vi "2636 EPSC Custom Pulse Sweep.vi"() -> ()   [LabVIEW 2023]
uses:
  <instrlib>/Keithley 2600 Series/Public/Channel.ctl
  <instrlib>/Keithley 2600 Series/Keithley 2600 Series.lvlib
  <userlib>/_OpenG.lib/time/time.llb/openg_time.lvlib
panel:
  out "Pulse Level Size":i32
  in  "Pulse Levels (V)":dbl[](array[numeric])=[1.0, 2.0, 4.0]
  in  "error in (no error)":errorcluster
  in  "Log Time After Pulses (s)":dbl=0.5 format="%#_13g"
  in  "Log Time Before Pulses (s)":dbl=0.5 format="%#_13g"
  in  "Auto Enable Output":bool=TRUE
  in  "Reset":bool=TRUE
  in  "Error Query":bool
  out "Pulsed IV Filename Out":path caption="Filename Out"
  in  "Pulsed IV Filename":path=path "C:/Data/pulse_I_V.lvm" caption="Filename"
  out "Pulse IV":cluster{"X":dbl[], "Y":dbl[]}[](graph)
  out "I_ds Log Filename Out":path caption="Filename Out"
  in  "I_ds Log Filename":path=path "C:/Data/I_ds_vs_time.lvm" caption="Filename"
  out "Data":dbl[](array[numeric])
  out "Result Chart":dynamicdata(graph)
  out "error out":errorcluster
  out "Complete?":bool
  out "Overflow?":bool
  in  "Stop":bool
  in  "Pulse Duration (s)":dbl=0.01
  in  "Post-Pulse Duration (s)":dbl=0.05
  in  "Pre-Pulse Duration (s)":dbl=0.05
  in  "Buffer size":u32=1024
  in  "Drain Source Channel":T1=enum."Channel B"
  in  "V_ds(V)":dbl=0.01
  in  "I_ds NPLC":dbl=0.1
  in  "I_ds Range (A)":dbl=1e-06
  in  "I pulse Range (A)":dbl=1e-06
  in  "I pulse NPLC":dbl=0.1
  in  "Pulse Channel":T1
  in  "2636 Address":refnum<visa-resource-name>="GPIB0::26::INSTR"
  # "Synaptic EPSC Custom Pulse Sweep (Three-terminal Devices)"
  # "by JHC (20250322)"
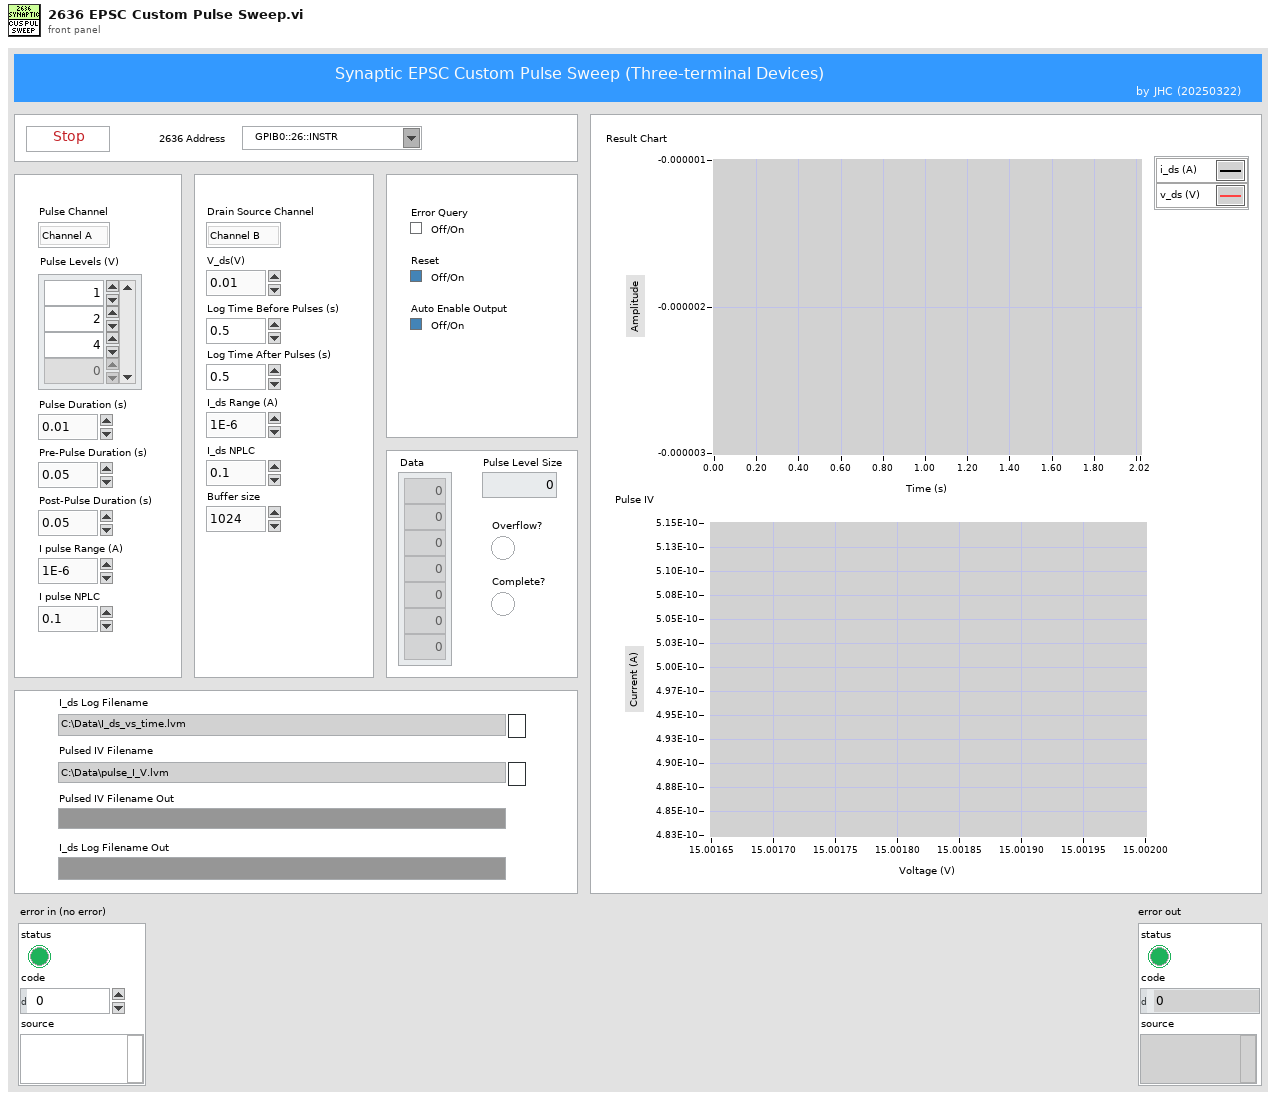
[diagram p1: front panel]
types:
  T1 = typedef "Keithley 2600 Series.lvlib/Channel.ctl" = enum32{"Channel A", "Channel B"}
  T2 = enum16{"None/Disconnect", "Digital I/O Trigger", "TSP-Link Trigger", "LAN Trigger", "Blender", "Timer Expired", "Front Panel Trigger", "Software Trigger", "SMU Sweeping", "SMU Armed", "SMU Source Complete", "SMU Measure Complete", "SMU Pulse Complete", "SMU Sweep Complete", "SMU Idle"}
  T3 = enum16{"Current", "Voltage", "IV", "Resistance", "Power"}
  T4 = enum32{"ASCII", "Real 32", "Real 64", "Single Precision Real", "Double Precision Real"}
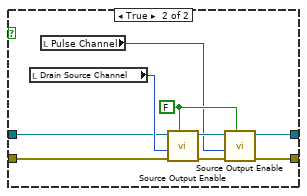
[diagram p2: hidden frame]
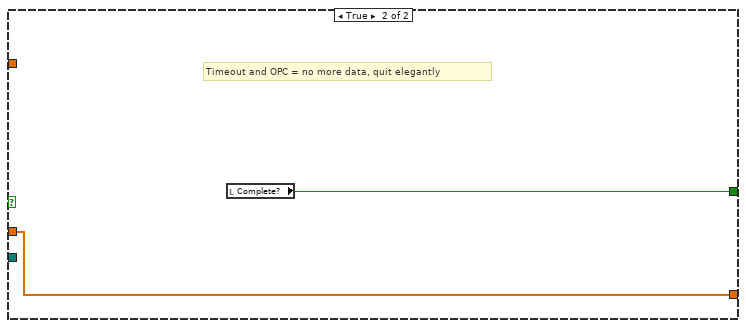
[diagram p5: hidden frame]
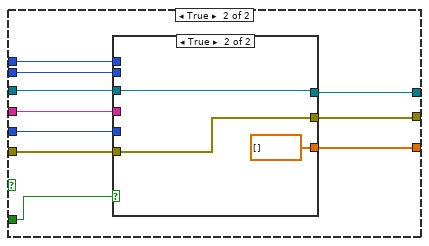
[diagram p8: hidden frame]
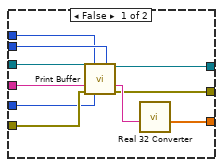
[diagram p9: hidden frame]
diagram:
  w19 = sgl[] [] ("Data Array Out")
  w22 = u16 1 items=["Channel A", "Channel B"] ("Channel (Channel A)")
  w23 = u16 0 items=["Channel A", "Channel B"] ("Channel (Channel A)")
  w39 = u16 0 items=["Current", "Voltage", "Resistance", "Power"] ("Function (Current)")
  w47 = u16 2 items=["Channel A", "Channel B", "Channels A & B", "User"] ("Screen (Channels A & B)")
  # "Wait 1s"
  # "Start Pulse SMU"
  # "Start DS SMU"
  n1 = call <instrlib>:"Initialize.vi"("Reset (True)"="Reset", "error in (no error)"="error in (no error)", "Error Query (False)"="Error Query", "ID Query (True)"=TRUE, "VISA resource name"="2636 Address") -> ("error out"=w2:errorcluster, "VISA resource name out"=w5:refnum<visa-resource-name>)  [unwired: 5 in]
  n2 = call <instrlib>:"Error Queue Clear.vi"("error in (no error)"=w2, "VISA resource name"=w5) -> ("error out"=w3:errorcluster, "VISA resource name out"=w4:refnum<visa-resource-name>)  [unwired: 6 in, 2 out]
  n3 = call <instrlib>:"Abort SMU Op.vi"("error in"=w3, "Channel (Channel A)"=w23, "VISA resource name"=w4) -> ("error out"=w24:errorcluster, "VISA resource name out"=w25:refnum<visa-resource-name>)  [unwired: 5 in, 2 out]
  n4 = call <instrlib>:"Abort SMU Op.vi"("error in"=w24, "Channel (Channel A)"=w22, "VISA resource name"=w25) -> ("error out"=w20:errorcluster, "VISA resource name out"=w21:refnum<visa-resource-name>)  [unwired: 5 in, 2 out]
  n5 = call <instrlib>:"Reset SMU.vi"("SMU B (No)"="Reset", "SMU A (No)"="Reset", "error in (no error)"=w20, "VISA resource name"=w21) -> ("error out"=w86:errorcluster, "VISA resource name out"=w87:refnum<visa-resource-name>)  [unwired: 4 in, 2 out]
  n6 = flat-sequence {
    tunnel: w87 -> [w122]
    tunnel: w86 -> [w121]
    tunnel: [w103] -> w85
    tunnel: [w102] -> w84
    tunnel: w85 -> [w145]
    tunnel: w84 -> [w146]
    tunnel: [w144] -> w83
    tunnel: [w143] -> w82
    tunnel: w83 -> [w187]
    tunnel: w82 -> [w185]
    tunnel: [w166] -> w81
    tunnel: [w165] -> w80
    tunnel: w81 -> [w267]
    tunnel: w80 -> [w266]
    tunnel: [w235] -> w79
    tunnel: [w234] -> w78
    tunnel: [w221] -> w77
    tunnel: w79 -> [w299]
    tunnel: w78 -> [w300]
    tunnel: w77 -> [w322]
    tunnel: [w303] -> w76
    tunnel: [w302] -> w75
    tunnel: w76 -> [w330]
    tunnel: w75 -> [w329]
    tunnel: [w326] -> w44
    tunnel: [w325] -> w43
    frame #0 {
      w110 = enum32{"Current", "Voltage"}."Current" ("Function (Current)")
      w111 = FALSE ("Autorange (On)")
      w91 = enum32{"Current", "Voltage"}."Voltage" ("Function (Current)")
      # "Init Pulse Gate Channel"
      n7 = local read "Pulse Levels (V)"() -> (w89:dbl[])
      n8 = call <instrlib>:"Source Function.vi"("Function (Current)"=w91, "error in (no error)"=w121, "Channel (Channel A)"="Pulse Channel", "VISA resource name"=w122) -> ("error out"=w123:errorcluster, "VISA resource name out"=w124:refnum<visa-resource-name>)  [unwired: 4 in, 2 out]
      n9 = call <instrlib>:"Source Level.vi"("Level (0.000)"=0.0, "Function (Current)"=w91, "error in (no error)"=w123, "Channel (Channel A)"="Pulse Channel", "VISA resource name"=w124) -> ("error out"=w119:errorcluster, "VISA resource name out"=w120:refnum<visa-resource-name>)  [unwired: 3 in, 2 out]
      n10 = Array Size(array=w89) -> (size(s)=→"Pulse Level Size":i32)
      n11 = Array Max & Min(array=w89) -> (max value=w90:dbl)  [unwired: 3 out]
      n12 = call <instrlib>:"Source Autorange.vi"("Autorange (On)"=w111, "Function (Current)"=w91, "error in (no error)"=w119, "Channel (Channel A)"="Pulse Channel", "VISA resource name"=w120) -> ("error out"=w117:errorcluster, "VISA resource name out"=w118:refnum<visa-resource-name>)  [unwired: 3 in, 2 out]
      n13 = call <instrlib>:"Source Autorange.vi"("Autorange (On)"=w111, "Function (Current)"=w110, "error in (no error)"=w117, "Channel (Channel A)"="Pulse Channel", "VISA resource name"=w118) -> ("error out"=w98:errorcluster, "VISA resource name out"=w100:refnum<visa-resource-name>)  [unwired: 3 in, 2 out]
      n14 = call <instrlib>:"Source Range.vi"("Range (1.000)"=w90, "Function (Current)"=w91, "error in (no error)"=w98, "Channel (Channel A)"="Pulse Channel", "VISA resource name"=w100) -> ("error out"=w97:errorcluster, "VISA resource name out"=w99:refnum<visa-resource-name>)  [unwired: 3 in, 2 out]
      n15 = call <instrlib>:"Measure NPLC.vi"("NPLC (1.000)"="I pulse NPLC", "error in (no error)"=w97, "Channel (Channel A)"="Pulse Channel", "VISA resource name"=w99) -> ("error out"=w115:errorcluster, "VISA resource name out"=w112:refnum<visa-resource-name>)  [unwired: 4 in, 2 out]
      n16 = call <instrlib>:"Measure Autorange.vi"("Autorange (On)"=w111, "Function (Current)"=w91, "error in (no error)"=w115, "Channel (Channel A)"="Pulse Channel", "VISA resource name"=w112) -> ("error out"=w114:errorcluster, "VISA resource name out"=w113:refnum<visa-resource-name>)  [unwired: 3 in, 2 out]
      n17 = call <instrlib>:"Measure Autorange.vi"("Autorange (On)"=w111, "Function (Current)"=w110, "error in (no error)"=w114, "Channel (Channel A)"="Pulse Channel", "VISA resource name"=w113) -> ("error out"=w96:errorcluster, "VISA resource name out"=w95:refnum<visa-resource-name>)  [unwired: 3 in, 2 out]
      n18 = call <instrlib>:"Measure Range.vi"("Range (1.000)"=w90, "Function (Current)"=w91, "error in (no error)"=w96, "Channel (Channel A)"="Pulse Channel", "VISA resource name"=w95) -> ("error out"=w93:errorcluster, "VISA resource name out"=w94:refnum<visa-resource-name>)  [unwired: 3 in, 2 out]
      n19 = call <instrlib>:"Measure Range.vi"("Range (1.000)"="I pulse Range (A)", "Function (Current)"=w110, "error in (no error)"=w93, "Channel (Channel A)"="Pulse Channel", "VISA resource name"=w94) -> ("error out"=w108:errorcluster, "VISA resource name out"=w107:refnum<visa-resource-name>)  [unwired: 3 in, 2 out]
      n20 = call <instrlib>:"Measure Sense Mode.vi"("error in (no error)"=w108, "Channel (Channel A)"="Pulse Channel", "VISA resource name"=w107) -> ("error out"=w105:errorcluster, "VISA resource name out"=w106:refnum<visa-resource-name>)  [unwired: 2 in, 5 out]
      n21 = call <instrlib>:"Measure Autozero.vi"("Autozero (Auto)"=enum32{"Off", "Once", "Auto"}."Once", "error in (no error)"=w105, "Channel (Channel A)"="Pulse Channel", "VISA resource name"=w106) -> ("error out"=w102:errorcluster, "VISA resource name out"=w103:refnum<visa-resource-name>)  [unwired: 1 in, 5 out]
    }
    frame #1 {
      w128 = 0.0 ("Interval (0.000)")
      w148 = enum32{"Current", "Voltage"}."Current" ("Function (Current)")
      w147 = FALSE ("Autorange (On)")
      w134 = enum32{"Current", "Voltage"}."Voltage" ("Function (Current)")
      # "Init Drain Source Channel"
      n22 = call <instrlib>:"Source Function.vi"("Function (Current)"=w134, "error in (no error)"=w146, "Channel (Channel A)"="Drain Source Channel", "VISA resource name"=w145) -> ("error out"=w162:errorcluster, "VISA resource name out"=w163:refnum<visa-resource-name>)  [unwired: 4 in, 2 out]
      n23 = call <instrlib>:"Source Level.vi"("Level (0.000)"="V_ds(V)", "Function (Current)"=w134, "error in (no error)"=w162, "Channel (Channel A)"="Drain Source Channel", "VISA resource name"=w163) -> ("error out"=w160:errorcluster, "VISA resource name out"=w161:refnum<visa-resource-name>)  [unwired: 3 in, 2 out]
      n24 = call <instrlib>:"Source Autorange.vi"("Autorange (On)"=w147, "Function (Current)"=w134, "error in (no error)"=w160, "Channel (Channel A)"="Drain Source Channel", "VISA resource name"=w161) -> ("error out"=w158:errorcluster, "VISA resource name out"=w159:refnum<visa-resource-name>)  [unwired: 3 in, 2 out]
      n25 = call <instrlib>:"Source Autorange.vi"("Autorange (On)"=w147, "Function (Current)"=w148, "error in (no error)"=w158, "Channel (Channel A)"="Drain Source Channel", "VISA resource name"=w159) -> ("error out"=w142:errorcluster, "VISA resource name out"=w139:refnum<visa-resource-name>)  [unwired: 3 in, 2 out]
      n26 = call <instrlib>:"Source Range.vi"("Range (1.000)"="V_ds(V)", "Function (Current)"=w134, "error in (no error)"=w142, "Channel (Channel A)"="Drain Source Channel", "VISA resource name"=w139) -> ("error out"=w141:errorcluster, "VISA resource name out"=w140:refnum<visa-resource-name>)  [unwired: 3 in, 2 out]
      n27 = call <instrlib>:"Measure NPLC.vi"("NPLC (1.000)"="I_ds NPLC", "error in (no error)"=w141, "Channel (Channel A)"="Drain Source Channel", "VISA resource name"=w140) -> ("error out"=w129:errorcluster, "VISA resource name out"=w130:refnum<visa-resource-name>)  [unwired: 4 in, 2 out]
      n28 = call <instrlib>:"Measure Interval.vi"("Interval (0.000)"=w128, "error in (no error)"=w129, "Channel (Channel A)"="Drain Source Channel", "VISA resource name"=w130) -> ("error out"=w132:errorcluster, "VISA resource name out"=w131:refnum<visa-resource-name>)  [unwired: 4 in, 2 out]
      n29 = call <instrlib>:"Measure Delay.vi"("Delay (0)"=w128, "error in (no error)"=w132, "Channel (Channel A)"="Drain Source Channel", "VISA resource name"=w131) -> ("error out"=w126:errorcluster, "VISA resource name out"=w127:refnum<visa-resource-name>)  [unwired: 4 in, 2 out]
      n30 = call <instrlib>:"Measure Autorange.vi"("Autorange (On)"=w147, "Function (Current)"=w134, "error in (no error)"=w126, "Channel (Channel A)"="Drain Source Channel", "VISA resource name"=w127) -> ("error out"=w156:errorcluster, "VISA resource name out"=w155:refnum<visa-resource-name>)  [unwired: 3 in, 2 out]
      n31 = call <instrlib>:"Measure Autorange.vi"("Autorange (On)"=w147, "Function (Current)"=w148, "error in (no error)"=w156, "Channel (Channel A)"="Drain Source Channel", "VISA resource name"=w155) -> ("error out"=w135:errorcluster, "VISA resource name out"=w136:refnum<visa-resource-name>)  [unwired: 3 in, 2 out]
      n32 = call <instrlib>:"Measure Range.vi"("Range (1.000)"="V_ds(V)", "Function (Current)"=w134, "error in (no error)"=w135, "Channel (Channel A)"="Drain Source Channel", "VISA resource name"=w136) -> ("error out"=w138:errorcluster, "VISA resource name out"=w137:refnum<visa-resource-name>)  [unwired: 3 in, 2 out]
      n33 = call <instrlib>:"Measure Range.vi"("Range (1.000)"="I_ds Range (A)", "Function (Current)"=w148, "error in (no error)"=w138, "VISA resource name"=w137) -> ("error out"=w153:errorcluster, "VISA resource name out"=w152:refnum<visa-resource-name>)  [unwired: 4 in, 2 out]
      n34 = call <instrlib>:"Measure Sense Mode.vi"("error in (no error)"=w153, "Channel (Channel A)"="Drain Source Channel", "VISA resource name"=w152) -> ("error out"=w150:errorcluster, "VISA resource name out"=w151:refnum<visa-resource-name>)  [unwired: 2 in, 5 out]
      n35 = call <instrlib>:"Measure Autozero.vi"("Autozero (Auto)"=enum32{"Off", "Once", "Auto"}."Once", "error in (no error)"=w150, "Channel (Channel A)"="Drain Source Channel", "VISA resource name"=w151) -> ("error out"=w144:errorcluster, "VISA resource name out"=w143:refnum<visa-resource-name>)  [unwired: 1 in, 5 out]
    }
    frame #2 {
      w179 = TRUE ("Append Mode (Off)")
      w178 = "v_ds" ("Buffer Name (buf)")
      w180 = TRUE ("Append Mode (Off)")
      w182 = "i_ds" ("Buffer Name (buf)")
      w191 = FALSE ("Collect Timestamps (Off)")
      w190 = "pulse_iv_table.v" ("Buffer Name (buf)")
      w189 = TRUE ("Append Mode (Off)")
      w188 = "pulse_iv_table.i" ("Buffer Name (buf)")
      # "set up circular buffer"
      # "A large size"
      # "Init Buffer"
      n36 = local read "Pulse Level Size"() -> (w164:i32)
      n37 = local read "Pulse Channel"() -> (w206:T1)
      n38 = VISA Write(VISA resource name=w185, write buffer="pulse_iv_table = {}\nds_iv_table = {}", error in (no error)=w187) -> (VISA resource name out=w192:refnum<visa-resource-name>, error out=w193:errorcluster)  [unwired: 1 out]
      n39 = call <instrlib>:"Error Query.vi"("error in (no error)"=w193, "VISA resource name"=w192) -> ("error out"=w205:errorcluster, "VISA resource name out"=w204:refnum<visa-resource-name>)  [unwired: 8 out]
      n40 = call <instrlib>:"Buffer Make Buffer.vi"("Capacity (1)"=w164, "Channel (Channel A)"=w206, "error in (no error)"=w205, "Buffer Name (buf)"=w188, "VISA resource name"=w204) -> ("error out"=w194:errorcluster, "VISA resource name out"=w195:refnum<visa-resource-name>)  [unwired: 1 in, 4 out]
      n41 = call <instrlib>:"Buffer Clear.vi"("error in (no error)"=w194, "Buffer Name"=w188, "VISA resource name"=w195) -> ("error out"=w197:errorcluster, "VISA resource name out"=w196:refnum<visa-resource-name>)  [unwired: 7 out]
      n42 = call <instrlib>:"Buffer Configure.vi"("Collect Timestamps (Off)"=w191, "error in (no error)"=w197, "Buffer Name"=w188, "Append Mode (Off)"=w189, "VISA resource name"=w196) -> ("error out"=w199:errorcluster, "VISA resource name out"=w198:refnum<visa-resource-name>)  [unwired: 2 in, 3 out]
      n43 = call <instrlib>:"Buffer Make Buffer.vi"("Capacity (1)"=w164, "Channel (Channel A)"=w206, "error in (no error)"=w199, "Buffer Name (buf)"=w190, "VISA resource name"=w198) -> ("error out"=w201:errorcluster, "VISA resource name out"=w200:refnum<visa-resource-name>)  [unwired: 1 in, 4 out]
      n44 = call <instrlib>:"Buffer Clear.vi"("error in (no error)"=w201, "Buffer Name"=w190, "VISA resource name"=w200) -> ("error out"=w203:errorcluster, "VISA resource name out"=w202:refnum<visa-resource-name>)  [unwired: 7 out]
      n45 = call <instrlib>:"Buffer Configure.vi"("Collect Source Values (Off)"=w191, "error in (no error)"=w203, "Buffer Name"=w190, "Append Mode (Off)"=w189, "VISA resource name"=w202) -> ("error out"=w212:errorcluster, "VISA resource name out"=w211:refnum<visa-resource-name>)  [unwired: 2 in, 3 out]
      n46 = local read "Drain Source Channel"() -> (w170:T1)
      n47 = call <instrlib>:"Buffer Make Buffer.vi"("Capacity (1)"="Buffer size", "Channel (Channel A)"=w170, "error in (no error)"=w212, "Buffer Name (buf)"=w182, "VISA resource name"=w211) -> ("error out"=w208:errorcluster, "VISA resource name out"=w207:refnum<visa-resource-name>)  [unwired: 1 in, 4 out]
      n48 = call <instrlib>:"Buffer Clear.vi"("error in (no error)"=w208, "Buffer Name"=w182, "VISA resource name"=w207) -> ("error out"=w210:errorcluster, "VISA resource name out"=w209:refnum<visa-resource-name>)  [unwired: 7 out]
      n49 = call <instrlib>:"Buffer Configure.vi"("Collect Timestamps (Off)"=w180, "error in (no error)"=w210, "Buffer Name"=w182, "Append Mode (Off)"=w180, "VISA resource name"=w209) -> ("error out"=w184:errorcluster, "VISA resource name out"=w183:refnum<visa-resource-name>)  [unwired: 2 in, 3 out]
      n50 = call <instrlib>:"Advanced Buffer Configuration.vi"("VISA resource name"=w183, "Enable Buffer Cache Mode (Disable)"=w180, "Buffer Name"=w182, "Buffer Fill Mode (Fill_Once)"=enum16{"FILL_ONCE", "FILL_WINDOW"}."FILL_WINDOW", "error in (no error)"=w184) -> ("VISA resource name out"=w168:refnum<visa-resource-name>, "error out"=w167:errorcluster)  [unwired: 9 in]
      n51 = call <instrlib>:"Buffer Make Buffer.vi"("Capacity (1)"="Buffer size", "Channel (Channel A)"=w170, "error in (no error)"=w167, "Buffer Name (buf)"=w178, "VISA resource name"=w168) -> ("error out"=w174:errorcluster, "VISA resource name out"=w175:refnum<visa-resource-name>)  [unwired: 1 in, 4 out]
      n52 = call <instrlib>:"Buffer Clear.vi"("error in (no error)"=w174, "Buffer Name"=w178, "VISA resource name"=w175) -> ("error out"=w172:errorcluster, "VISA resource name out"=w173:refnum<visa-resource-name>)  [unwired: 7 out]
      n53 = call <instrlib>:"Buffer Configure.vi"("Collect Timestamps (Off)"=w179, "error in (no error)"=w172, "Buffer Name"=w178, "Append Mode (Off)"=w179, "VISA resource name"=w173) -> ("error out"=w176:errorcluster, "VISA resource name out"=w177:refnum<visa-resource-name>)  [unwired: 2 in, 3 out]
      n54 = call <instrlib>:"Advanced Buffer Configuration.vi"("VISA resource name"=w177, "Enable Buffer Cache Mode (Disable)"=w179, "Buffer Name"=w178, "Buffer Fill Mode (Fill_Once)"=enum16{"FILL_ONCE", "FILL_WINDOW"}."FILL_WINDOW", "error in (no error)"=w176) -> ("VISA resource name out"=w165:refnum<visa-resource-name>, "error out"=w166:errorcluster)  [unwired: 9 in]
    }
    frame #3 {
      w225 = u32 4 ("Timer Number (1)")
      w238 = u32 1 ("Timer Number (1)")
      w249 = u32 3 ("Timer Number (1)")
      w272 = u32 2 ("Timer Number (1)")
      # "SMU Armed when timer4 expires"
      # "Trigger timer4 when the SMU Sweeping, only once"
      # "Trigger timer1 when the SMU Armed, repeat N times"
      # "Trigger end pulse after timer3 expired"
      # "Configure measure action (default is 0) to start after source immediately"
      # "set source pulse level and end pusle idle"
      # "Trigger timer3 when the SMU source pulse level"
      # "Create a fixed level voltage sweep"
      # "Configure source action to start after timer2 expired"
      # "Trigger timer2 when timer1 expired or first run."
      # "Init Trigger Model (Pulse Channel)"
      n55 = Array To Spreadsheet String(delimiter (Tab)=",", array="Pulse Levels (V)", 3:"%f" ("format string")) -> (spreadsheet string=w215:string)
      n56 = local read "Pulse Channel"() -> (w221:T1)
      n57 = Pick Line(multi-line string="smua\nsmub", line index=w221) -> (output string=w233:string)  [unwired: 1 in]
      n58 = Format Into String(format string="%s.trigger.source.listv({%s})\\n", w233, w215) -> (resulting string=w270:string)  [unwired: 2 in, 1 out]
      n59 = call <instrlib>:"Format Event ID.vi"("Channel (Channel A)"=w221, "Event Type (None)"=T2."SMU Sweeping") -> ("Event ID"=w229:string)  [unwired: 8 in, 1 out]
      n60 = Format Into String(format string="%s.trigger.source.action = %s.ENABLE\n%s.trigger.endpulse.action = %s.SOURCE_IDLE", initial string=w270, w233, w233, w233, w233) -> (resulting string=w265:string)  [unwired: 1 in, 1 out]
      n61 = VISA Write(VISA resource name=w266, write buffer=w265, error in (no error)=w267) -> (VISA resource name out=w231:refnum<visa-resource-name>, error out=w230:errorcluster)  [unwired: 1 out]
      n62 = call <instrlib>:"Config Timer.vi"("VISA resource name"=w231, "Delay (1e-3)"="Log Time Before Pulses (s)", "Timer Number (1)"=w225, "error in"=w230, "Input Event"=w229) -> ("VISA resource name out"=w227:refnum<visa-resource-name>, "error out"=w223:errorcluster)  [unwired: 7 in, 2 out]
      n63 = call <instrlib>:"Format Event ID.vi"("Event Module # (1)"=w225, "Event Type (None)"=T2."Timer Expired") -> ("Event ID"=w224:string)  [unwired: 8 in, 1 out]
      n64 = call <instrlib>:"Config Arm Event.vi"("Arm Input Event"=w224, "error in"=w223, "Channel (Channel A)"=w221, "VISA resource name"=w227) -> ("error out"=w219:errorcluster, "VISA resource name out"=w218:refnum<visa-resource-name>)  [unwired: 4 in, 2 out]
      n65 = local read "Pulse Level Size"() -> (w213:i32)
      n66 = call <instrlib>:"Format Event ID.vi"("Channel (Channel A)"=w221, "Event Type (None)"=T2."SMU Armed") -> ("Event ID"=w220:string)  [unwired: 8 in, 1 out]
      n67 = local read "Pre-Pulse Duration (s)"() -> (w246:dbl)
      n68 = local read "Pulse Duration (s)"() -> (w247:dbl)
      n69 = Decrement(x=w213) -> (x-1=w239:i32)
      n70 = Compound Arithmetic op=ADD(w247, w246, "Post-Pulse Duration (s)") -> (w244:dbl)
      n71 = call <instrlib>:"Config Timer.vi"("VISA resource name"=w218, "Count (1)"=w239, "Delay (1e-3)"=w244, "Timer Number (1)"=w238, "Passthrough (Off)"=TRUE, "error in"=w219, "Input Event"=w220) -> ("VISA resource name out"=w240:refnum<visa-resource-name>, "error out"=w241:errorcluster)  [unwired: 5 in, 2 out]
      n72 = call <instrlib>:"Format Event ID.vi"("Event Module # (1)"=w238, "Event Type (None)"=T2."Timer Expired") -> ("Event ID"=w276:string)  [unwired: 8 in, 1 out]
      n73 = call <instrlib>:"Config Timer.vi"("VISA resource name"=w240, "Delay (1e-3)"="Pre-Pulse Duration (s)", "Timer Number (1)"=w272, "error in"=w241, "Input Event"=w276) -> ("VISA resource name out"=w275:refnum<visa-resource-name>, "error out"=w274:errorcluster)  [unwired: 7 in, 2 out]
      n74 = call <instrlib>:"Format Event ID.vi"("Event Module # (1)"=w272, "Event Type (None)"=T2."Timer Expired") -> ("Event ID"=w271:string)  [unwired: 8 in, 1 out]
      n75 = call <instrlib>:"Config Source Event.vi"("Input Event"=w271, "error in"=w274, "Channel (Channel A)"=w221, "VISA resource name"=w275) -> ("error out"=w260:errorcluster, "VISA resource name out"=w261:refnum<visa-resource-name>)  [unwired: 4 in, 2 out]
      n76 = call <instrlib>:"Format Event ID.vi"("Channel (Channel A)"=w221, "Event Type (None)"=T2."SMU Source Complete") -> ("Event ID"=w263:string)  [unwired: 8 in, 1 out]
      n77 = call <instrlib>:"Config Timer.vi"("VISA resource name"=w261, "Delay (1e-3)"="Pulse Duration (s)", "Timer Number (1)"=w249, "error in"=w260, "Input Event"=w263) -> ("VISA resource name out"=w259:refnum<visa-resource-name>, "error out"=w258:errorcluster)  [unwired: 7 in, 2 out]
      n78 = call <instrlib>:"Config Measure Event.vi"("VISA resource name"=w259, "Configure Measurement (Disable)"=enum8{"DISABLE", "ENABLE", "ASYNC"}."ENABLE", "Buffer 1"="pulse_iv_table.i" ("Buffer Name (buf)"), "Buffer 2"="pulse_iv_table.v" ("Buffer Name (buf)"), "Channel (Channel A)"=w221, "Function (Current)"=T3."IV", "error in"=w258, "Measure Input Event"="0") -> ("VISA resource name out"=w252:refnum<visa-resource-name>, "error out"=w251:errorcluster)  [unwired: 4 in, 2 out]
      n79 = call <instrlib>:"Format Event ID.vi"("Event Module # (1)"=w249, "Event Type (None)"=T2."Timer Expired") -> ("Event ID"=w248:string)  [unwired: 8 in, 1 out]
      n80 = call <instrlib>:"Config End Pulse Event.vi"("Input Event"=w248, "error in"=w251, "Channel (Channel A)"=w221, "VISA resource name"=w252) -> ("error out"=w237:errorcluster, "VISA resource name out"=w236:refnum<visa-resource-name>)  [unwired: 4 in, 2 out]
      n81 = call <instrlib>:"Config Layer Count.vi"("Trigger Count (1)"=w213, "Arm Count (1)"=u32 1 ("Trigger Count (1)"), "error in"=w237, "Channel (Channel A)"=w221, "VISA resource name"=w236) -> ("error out"=w234:errorcluster, "VISA resource name out"=w235:refnum<visa-resource-name>)  [unwired: 3 in, 2 out]
    }
    frame #4 {
      w284 = u32 5 ("Timer Number (1)")
      w312 = u32 1 ("Blender Number (1)")
      # "BUG from Driver: if Async, measure.Y is not set"
      # "No trigger, start\nasync measure after SMU Armed, as fast as possible"
      # "Trigger timer5 when Pulse SMU Idle\nto keep measure for a while"
      # "Blend two events from Pulse SMU to trigger DS SMU Source action\nDS SMU Source start when Pulse SMU start sweeping\nWhen Pulse SMU become idle, DS SMU source again and stop"
      # "set source level, and hold"
      # "Create a fixed level voltage sweep"
      # "Init Trigger Model (Drain Source Channel)"
      n82 = local read "Drain Source Channel"() -> (w305:T1)
      n83 = local read "V_ds(V)"() -> (w316:dbl)
      n84 = Pick Line(multi-line string="smua\nsmub", line index=w305) -> (output string=w292:string)  [unwired: 1 in]
      n85 = Format Into String(format string="%s.trigger.source.listv({%f})\\n", w292, w316) -> (resulting string=w319:string)  [unwired: 2 in, 1 out]
      n86 = Format Into String(format string="%s.trigger.source.action = %s.ENABLE\n%s.trigger.endpulse.action = %s.SOURCE_HOLD", initial string=w319, w292, w292, w292, w292) -> (resulting string=w298:string)  [unwired: 1 in, 1 out]
      n87 = VISA Write(VISA resource name=w299, write buffer=w298, error in (no error)=w300) -> (VISA resource name out=w288:refnum<visa-resource-name>, error out=w289:errorcluster)  [unwired: 1 out]
      n88 = call <instrlib>:"Format Event ID.vi"("Channel (Channel A)"=w322, "Event Type (None)"=T2."SMU Sweeping") -> ("Event ID"=w283:string)  [unwired: 8 in, 1 out]
      n89 = call <instrlib>:"Format Event ID.vi"("Channel (Channel A)"=w322, "Event Type (None)"=T2."SMU Idle") -> ("Event ID"=w286:string)  [unwired: 8 in, 1 out]
      n90 = call <instrlib>:"Config Timer.vi"("VISA resource name"=w288, "Delay (1e-3)"="Log Time After Pulses (s)", "Timer Number (1)"=w284, "error in"=w289, "Input Event"=w286) -> ("VISA resource name out"=w280:refnum<visa-resource-name>, "error out"=w281:errorcluster)  [unwired: 7 in, 2 out]
      n91 = call <instrlib>:"Format Event ID.vi"("Event Module # (1)"=w284, "Event Type (None)"=T2."Timer Expired") -> ("Event ID"=w282:string)  [unwired: 8 in, 1 out]
      n92 = call <instrlib>:"Config Event Blender.vi"("VISA resource name"=w280, "Input Event 1"=w282, "Input Event 2"=w283, "Blender Number (1)"=w312, "Blend Type (OR)"=enum16{"OR", "AND"}."OR", "error in"=w281) -> ("VISA resource name out"=w314:refnum<visa-resource-name>, "error out"=w315:errorcluster)  [unwired: 6 in, 2 out]
      n93 = call <instrlib>:"Format Event ID.vi"("Event Module # (1)"=w312, "Event Type (None)"=T2."Blender") -> ("Event ID"=w311:string)  [unwired: 8 in, 1 out]
      n94 = call <instrlib>:"Config Source Event.vi"("Input Event"=w311, "error in"=w315, "Channel (Channel A)"=w305, "VISA resource name"=w314) -> ("error out"=w308:errorcluster, "VISA resource name out"=w309:refnum<visa-resource-name>)  [unwired: 4 in, 2 out]
      n95 = call <instrlib>:"Config Measure Event.vi"("VISA resource name"=w309, "Configure Measurement (Disable)"=enum8{"DISABLE", "ENABLE", "ASYNC"}."ENABLE", "Buffer 1"="i_ds" ("Buffer Name (buf)"), "Buffer 2"="v_ds" ("Buffer Name (buf)"), "Channel (Channel A)"=w305, "Function (Current)"=T3."IV", "error in"=w308) -> ("VISA resource name out"=w294:refnum<visa-resource-name>, "error out"=w295:errorcluster)  [unwired: 5 in, 2 out]
      n96 = Format Into String(format string="%s.trigger.measure.action = %s.ASYNC", w292, w292) -> (resulting string=w291:string)  [unwired: 2 in, 1 out]
      n97 = VISA Write(VISA resource name=w294, write buffer=w291, error in (no error)=w295) -> (VISA resource name out=w297:refnum<visa-resource-name>, error out=w296:errorcluster)  [unwired: 1 out]
      n98 = call <instrlib>:"Config Layer Count.vi"("Trigger Count (1)"=u32 2 ("Arm Count (1)"), "Arm Count (1)"=u32 1, "error in"=w296, "Channel (Channel A)"=w305, "VISA resource name"=w297) -> ("error out"=w302:errorcluster, "VISA resource name out"=w303:refnum<visa-resource-name>)  [unwired: 3 in, 2 out]
    }
    frame #5 {
      # "Other init jobs"
      n99 = call <instrlib>:"Data Output Format.vi"("ASCII Precision (6)"=6, "error in (no error)"=w329, "Data Format (ASCII)"=T4."Real 32", "VISA resource name"=w330) -> ("error out"=w325:errorcluster, "VISA resource name out"=w326:refnum<visa-resource-name>)  [unwired: 4 in, 2 out]
    }
  }
  n100 = local read "Pulse Channel"() -> (w41:T1)
  n101 = local read "Drain Source Channel"() -> (w40:T1)
  n102 = call <instrlib>:"Display Screen.vi"("Screen (Channels A & B)"=w47, "error in (no error)"=w43, "VISA resource name"=w44) -> ("error out"=w50:errorcluster, "Node Out"=w49:string, "VISA resource name out"=w48:refnum<visa-resource-name>)  [unwired: 5 in, 1 out]
  n103 = call <instrlib>:"Display Measure Function.vi"("Function (Current)"=w39, "error in (no error)"=w50, "Channel (Channel A)"=w41, "Node In"=w49, "VISA resource name"=w48) -> ("error out"=w46:errorcluster, "VISA resource name out"=w45:refnum<visa-resource-name>)  [unwired: 3 in, 2 out]
  n104 = control-ref of="Overflow?"() -> (w36:refnum<vi>)
  n105 = control-ref of="Complete?"() -> (w35:refnum<vi>)
  n106 = control-ref of="Stop"() -> (w30:refnum<vi>)
  n107 = call <instrlib>:"Display Measure Function.vi"("Function (Current)"=w39, "error in (no error)"=w46, "Channel (Channel A)"=w40, "VISA resource name"=w45) -> ("error out"=w42:errorcluster, "VISA resource name out"=w38:refnum<visa-resource-name>)  [unwired: 4 in, 2 out]
  n108 = Build Array(w36, w35, w30) -> (w34:refnum<vi>[])
  n109 = case shown="True" "Auto Enable Output" {
    tunnel: [w331 w341] -> w9
    tunnel: [w332 w340] -> w10
    tunnel: w42 -> [w331 w336]
    tunnel: w41 -> [_ w335]
    tunnel: w40 -> [_ w334]
    tunnel: w38 -> [w332 w333]
    frame False {
    }
    frame True {
      w337 = TRUE ("Output (Off)")
      n110 = call <instrlib>:"Source Output Enable.vi"("Output (Off)"=w337, "error in (no error)"=w336, "Channel (Channel A)"=w334, "VISA resource name"=w333) -> ("error out"=w339:errorcluster, "VISA resource name out"=w338:refnum<visa-resource-name>)  [unwired: 4 in, 2 out]
      n111 = call <instrlib>:"Source Output Enable.vi"("Output (Off)"=w337, "error in (no error)"=w339, "Channel (Channel A)"=w335, "VISA resource name"=w338) -> ("error out"=w341:errorcluster, "VISA resource name out"=w340:refnum<visa-resource-name>)  [unwired: 4 in, 2 out]
    }
  }
  n112 = for {
    tunnel: w34 -> [w343] mode=indexing
    tunnel: [w342] -> w31
    # "Init GUI"
    n113 = invoke class="Bool (strict)" method="Reinit To Default"(reference=w343) -> (error out=w342:errorcluster)  [unwired: 2 in, 2 out]
  }
  n114 = call <userlib>:"Wait (ms)__ogtk.vi"("error in (no error)"=w9, "milliseconds to wait"=u32 1000) -> ("error out"=w8:errorcluster)  [unwired: 8 in, 1 out]
  n115 = call <instrlib>:"Initiate Sweep.vi"("error in"=w8, "Channel (Channel A)"=w40, "VISA resource name"=w10) -> ("error out"=w70:errorcluster, "VISA resource name out"=w71:refnum<visa-resource-name>)  [unwired: 5 in, 2 out]
  n116 = Obtain Queue(max queue size (-1, unlimited)=1024, name (unnamed)="data_q", element data type=w19, error in (no error)=w42) -> (queue out=w57:refnum<queue>, error out=w32:errorcluster)  [unwired: 1 in, 1 out]
  n117 = Format Into String(format string="%s, %s, %s", "i_ds" ("Buffer Name(s)"), "i_ds.timestamps" ("Buffer Name(s)"), "v_ds" ("Buffer Name(s)")) -> (resulting string=w74:string)  [unwired: 2 in, 1 out]
  n118 = call <instrlib>:"Initiate Sweep.vi"("error in"=w70, "Channel (Channel A)"=w41, "VISA resource name"=w71) -> ("error out"=w73:errorcluster, "VISA resource name out"=w72:refnum<visa-resource-name>)  [unwired: 5 in, 2 out]
  n119 = Merge Errors(w32, w31) -> (w33:errorcluster)
  n120 = while {
    tunnel: w57 -> [w355]
    tunnel: "I_ds Log Filename" -> [w351]
    tunnel: w33 -> [w354]
    tunnel: [w350] -> w29
    shift-right: [w344] -> w15
    shift-left: w19 -> [w345]
    stop <- w348 stop-if-true
    # "Plot and save I_ds and v_ds"
    n121 = Dequeue Element(queue=w355, timeout in ms (-1)=500, error in (no error)=w354) -> (queue out=w350:refnum<queue>, element=w352:sgl[], timed out?=w353:bool, error out=w347:errorcluster)
    n122 = case shown="False" w353 {
      tunnel: w352 -> [w358 _]
      tunnel: w351 -> [w367 _]
      tunnel: [FALSE ("Operation Complete") w380] -> w346
      tunnel: w345 -> [w359 w379]
      tunnel: [w357 w379] -> w344
      frame False {
        n123 = Decimate 1D Array(w358) -> (w364:sgl[], w363:sgl[], w362:sgl[])
        n124 = for {
          tunnel: [w376] -> w366
          tunnel: [w371] -> w361 mode=indexing
          tunnel: w364 -> [w370] mode=indexing
          tunnel: w363 -> [w369] mode=indexing
          tunnel: w362 -> [w374] mode=indexing
          n125 = To Time Stamp(1:w369) -> (0:w375:timestamp)
          n126 = Build Array(w370) -> (w373:sgl[])
          n127 = Build Array(w374) -> (w372:sgl[])
          n128 = Build Array(w369, w370, w374) -> (w371:sgl[])
          "Data" <- w371
          n129 = Bundle By Name("Y"=w373, "t0"=w375) -> (w378:waveform(sgl))  [unwired: 1 in]
          n130 = Bundle By Name("Y"=w372, "t0"=w375) -> (w377:waveform(sgl))  [unwired: 1 in]
          n131 = Merge Signals(w378, w377) -> (w376:dynamicdata)
        }
        "Result Chart" <- w366
        n132 = Build Array (concatenate)(w359, w358) -> (w357:sgl[])
        n133 = call "Convert to Dynamic Data3"("2D Array"=w361) -> ("Dynamic Data Type"=w365:dynamicdata)  [unwired: 3 in]
        n134 = call "Write To Measurement File"("Signals"=w365, "Filename"=w367) -> ("Filename Out"=→"I_ds Log Filename Out":path)  [unwired: 15 in, 2 out]
      }
      frame True {
        # "Timeout and OPC = no more data, quit elegantly"
        n135 = local read "Complete?"() -> (w380:bool)
      }
    }
    n136 = local read "Stop"() -> (w349:bool)
    n137 = Compound Arithmetic op=OR(w346, w349, w347) -> (w348:bool)
  }
  n138 = while {
    tunnel: w72 -> [w389]
    tunnel: w73 -> [w388]
    shift-right: [w383] -> _
    shift-left: u32 1 ("Start Index (1)") -> [w382]
    tunnel: w74 -> [w405]
    tunnel: "tostring(i_ds.next), tostring(v_ds.next)" ("format string") -> [w403]
    tunnel: w57 -> [w387]
    tunnel: [w402] -> w61
    tunnel: [w386] -> w60
    tunnel: [w390] -> w53
    stop <- w391 stop-if-true
    # "Fetch buffer data and parse dataframes"
    n139 = Wait (ms)(milliseconds to wait=u32 100) -> ()  [unwired: 1 out]
    n140 = VISA Write(VISA resource name=w389, write buffer="*OPC", error in (no error)=w388) -> (VISA resource name out=w401:refnum<visa-resource-name>, error out=w400:errorcluster)  [unwired: 1 out]
    n141 = call <instrlib>:"ESR.vi"("error in (no error)"=w400, "VISA resource name"=w401) -> ("error out"=w395:errorcluster, "ESR"=w399:u8, "VISA resource name out"=w394:refnum<visa-resource-name>)  [unwired: 5 in, 2 out]
    n142 = And(x=w399, y=u8 1) -> (x .and. y?=w398:u8)
    n143 = Not Equal To 0?(x=w398) -> (x != 0?=w390:bool)
    "Complete?" <- w390
    n144 = call <instrlib>:"Print.vi"("Byte Count (1024)"=u32 256, "error in (no error)"=w395, "Input"=w403, "VISA resource name"=w394) -> ("error out"=w412:errorcluster, "Output"=w414:string, "VISA resource name out"=w409:refnum<visa-resource-name>)  [unwired: 3 in, 2 out]
    n145 = Scan From String(format string="%d %d", input string=w414, error in=w412) -> (error out=w408:errorcluster, output 1=w411:i32, output 2=w410:i32)  [unwired: 3 in, 2 out]
    n146 = Max & Min(x=w411, y=w410) -> (min(x,y)=w383:i32)  [unwired: 1 out]
    n147 = Decrement(x=w383) -> (x-1=w393:i32)
    n148 = Greater Or Equal?(x=w383, y=w382) -> (x >= y?=w407:bool)
    n149 = Equal?(x=w383, y=w382) -> (x = y?=w381:bool)
    n150 = case shown="False" w407 {
      tunnel: w405 -> [w421 w448]
      tunnel: w409 -> [w424 w447]
      tunnel: w408 -> [w425 w446]
      tunnel: w393 -> [w431 w445]
      tunnel: w382 -> [w438 w444]
      tunnel: u32 4096 ("Byte Count (1024)") -> [w437 w443]
      tunnel: [w427 w442] -> w385
      tunnel: [w420 w440] -> w386
      tunnel: [w419 w441] -> w402
      tunnel: w381 -> [_ w439]
      frame False {
        n151 = VISA Write(VISA resource name=w424, write buffer="i_ds.clearcache()\nv_ds.clearcache()" ("format string"), error in (no error)=w425) -> (VISA resource name out=w423:refnum<visa-resource-name>, error out=w422:errorcluster)  [unwired: 1 out]
        n152 = local read "Buffer size"() -> (w436:u32)
        n153 = call <instrlib>:"Print Buffer.vi"("VISA resource name"=w423, "Start Index (1)"=w438, "End Index (1)"=w436, "Buffer Name(s)"=w421, "error in (no error)"=w422, "Byte Count (1024)"=w437) -> ("VISA resource name out"=w434:refnum<visa-resource-name>, "Buffer Data"=w435:string, "error out"=w433:errorcluster)  [unwired: 5 in, 2 out]
        n154 = call <instrlib>:"Real 32 Converter.vi"("Data In"=w435) -> ("Data Array Out"=w429:sgl[])  [unwired: 10 in]
        n155 = call <instrlib>:"Print Buffer.vi"("VISA resource name"=w434, "Start Index (1)"=u32 1, "End Index (1)"=w431, "Buffer Name(s)"=w421, "error in (no error)"=w433) -> ("VISA resource name out"=w419:refnum<visa-resource-name>, "Buffer Data"=w430:string, "error out"=w420:errorcluster)  [unwired: 6 in, 2 out]
        n156 = call <instrlib>:"Real 32 Converter.vi"("Data In"=w430) -> ("Data Array Out"=w428:sgl[])  [unwired: 10 in]
        n157 = Build Array (concatenate)(w429, w428) -> (w427:sgl[])
      }
      frame True {
        n158 = case shown="True" w439 {
          tunnel: w448 -> [w458 _]
          tunnel: w447 -> [w457 w461]
          tunnel: w446 -> [w456 w460]
          tunnel: w445 -> [w455 _]
          tunnel: w444 -> [w454 _]
          tunnel: w443 -> [w453 _]
          tunnel: [w451 sgl[] [] ("Data Array Out")] -> w442
          tunnel: [w450 w461] -> w441
          tunnel: [w449 w460] -> w440
          frame False {
            n159 = call <instrlib>:"Print Buffer.vi"("VISA resource name"=w457, "Start Index (1)"=w454, "End Index (1)"=w455, "Buffer Name(s)"=w458, "error in (no error)"=w456, "Byte Count (1024)"=w453) -> ("VISA resource name out"=w450:refnum<visa-resource-name>, "Buffer Data"=w452:string, "error out"=w449:errorcluster)  [unwired: 5 in, 2 out]
            n160 = call <instrlib>:"Real 32 Converter.vi"("Data In"=w452) -> ("Data Array Out"=w451:sgl[])  [unwired: 10 in]
          }
          frame True {
          }
        }
      }
    }
    n161 = Empty Array?(array=w385) -> (empty?=w384:bool)
    n162 = case shown="False" w384 {
      tunnel: w387 -> [w417 _]
      tunnel: w385 -> [w416 _]
      frame False {
        n163 = Lossy Enqueue Element(queue=w417, element=w416) -> (overflow?=→"Overflow?":bool)  [unwired: 1 in, 3 out]
      }
      frame True {
      }
    }
    n164 = Or(x=w390, y="Stop") -> (x .or. y?=w391:bool)
  }
  n165 = Release Queue(queue=w29) -> (error out=w26:errorcluster)  [unwired: 2 in, 2 out]
  n166 = Decimate 1D Array(w15) -> (w18:sgl[], w17:sgl[], w16:sgl[])
  n167 = for {
    tunnel: w18 -> [w467] mode=indexing
    tunnel: w17 -> [w463] mode=indexing
    tunnel: w16 -> [w466] mode=indexing
    n168 = To Time Stamp(1:w463) -> (0:w468:timestamp)
    n169 = Build Array(w467) -> (w465:sgl[])
    n170 = Build Array(w466) -> (w464:sgl[])
    n171 = Bundle By Name("Y"=w465, "t0"=w468) -> (w470:waveform(sgl))  [unwired: 1 in]
    n172 = Bundle By Name("Y"=w464, "t0"=w468) -> (w469:waveform(sgl))  [unwired: 1 in]
    n173 = Merge Signals(w470, w469) -> (w462:dynamicdata)
    n174 = local write "Result Chart"(w462) -> ()
  }
  n175 = case shown="False" w53 {
    tunnel: w61 -> [w478 w480]
    tunnel: w60 -> [w477 w479]
    tunnel: [w472 w480] -> w59
    tunnel: [w471 w479] -> w58
    frame False {
      w473 = u16 1 items=["Channel A", "Channel B"] ("Channel (Channel A)")
      w474 = u16 0 items=["Channel A", "Channel B"] ("Channel (Channel A)")
      # "Abort Operation"
      n176 = call <instrlib>:"Abort SMU Op.vi"("error in"=w477, "Channel (Channel A)"=w474, "VISA resource name"=w478) -> ("error out"=w475:errorcluster, "VISA resource name out"=w476:refnum<visa-resource-name>)  [unwired: 5 in, 2 out]
      n177 = call <instrlib>:"Abort SMU Op.vi"("error in"=w475, "Channel (Channel A)"=w473, "VISA resource name"=w476) -> ("error out"=w471:errorcluster, "VISA resource name out"=w472:refnum<visa-resource-name>)  [unwired: 5 in, 2 out]
    }
    frame True {
      # "Operation Completed"
    }
  }
  n178 = local read "Auto Enable Output"() -> (w11:bool)
  n179 = case shown="False" w11 {
    tunnel: w59 -> [w482 w486]
    tunnel: w58 -> [w481 w485]
    tunnel: [w481 w484] -> w55
    tunnel: [w482 w483] -> w54
    frame False {
    }
    frame True {
      w491 = FALSE ("Output (Off)")
      n180 = local read "Drain Source Channel"() -> (w488:T1)
      n181 = local read "Pulse Channel"() -> (w487:T1)
      n182 = call <instrlib>:"Source Output Enable.vi"("Output (Off)"=w491, "error in (no error)"=w485, "Channel (Channel A)"=w488, "VISA resource name"=w486) -> ("error out"=w489:errorcluster, "VISA resource name out"=w490:refnum<visa-resource-name>)  [unwired: 4 in, 2 out]
      n183 = call <instrlib>:"Source Output Enable.vi"("Output (Off)"=w491, "error in (no error)"=w489, "Channel (Channel A)"=w487, "VISA resource name"=w490) -> ("error out"=w484:errorcluster, "VISA resource name out"=w483:refnum<visa-resource-name>)  [unwired: 4 in, 2 out]
    }
  }
  n184 = case shown="True" w53 {
    tunnel: w55 -> [w492 w511]
    tunnel: w54 -> [w493 w510]
    tunnel: [w492 w499] -> w52
    tunnel: [w493 w505] -> w51
    frame False {
      # "Operation Aborted, do nothing"
    }
    frame True {
      # "Plot and save Pulsed IV (single point)"
      n185 = local read "Pulse Level Size"() -> (w507:i32)
      n186 = call <instrlib>:"Print Buffer.vi"("VISA resource name"=w510, "End Index (1)"=w507, "Buffer Name(s)"="pulse_iv_table.v, pulse_iv_table.i" ("Buffer Name (buf)"), "error in (no error)"=w511, "Byte Count (1024)"=u32 4096) -> ("VISA resource name out"=w505:refnum<visa-resource-name>, "Buffer Data"=w506:string, "error out"=w500:errorcluster)  [unwired: 6 in, 2 out]
      n187 = call <instrlib>:"Real 32 Converter.vi"("Data In"=w506) -> ("Data Array Out"=w504:sgl[])  [unwired: 10 in]
      n188 = Decimate 1D Array(w504) -> (w503:sgl[], w502:sgl[])
      n189 = call "Convert to Dynamic Data2"("Array"=w502) -> ("Dynamic Data Type"=w497:dynamicdata)  [unwired: 3 in]
      n190 = call "Convert to Dynamic Data"("Array"=w503) -> ("Dynamic Data Type"=w498:dynamicdata)  [unwired: 3 in]
      n191 = Merge Signals(w498, w497) -> (w494:dynamicdata)
      n192 = call "Build XY Graph"("error in (no error)"=w500, "Y Input"=w497, "X Input"=w498) -> ("error out"=w499:errorcluster, "XY Graph"=→"Pulse IV":cluster{"X":dbl[], "Y":dbl[]}[])  [unwired: 7 in]
      n193 = call "Write To Measurement File2"("Signals"=w494, "Filename"="Pulsed IV Filename") -> ("Filename Out"=→"Pulsed IV Filename Out":path)  [unwired: 15 in, 2 out]
    }
  }
  n194 = call <instrlib>:"Close.vi"("error in (no error)"=w52, "VISA resource name"=w51) -> ("error out"=w28:errorcluster)  [unwired: 9 in]
  n195 = Merge Errors(w28, w26) -> (→"error out":errorcluster)
